vi "optical_grab2.vi"() -> ()   [LabVIEW 2025]
uses:
  <vilib>/vision/driver/NI_Vision_Acquisition_Software.lvlib
  <resource>/objmgr/imaqdx.rc
panel:
  in  "Stop 2":bool
  out "Time bw Frames":u32
  out "max value":u16
  out "Image Pixels (U16)":u16[][](array[numeric])
  out "Image Preview":T1(plugin-control)
  out "error out":errorcluster
  out "FPS":u32
  in  "Output Folder":path=path "../data/raw/test_6"
  in  "Stop":bool
  in  "Camera Name":refnum<k21> caption="IMAQdx Session"
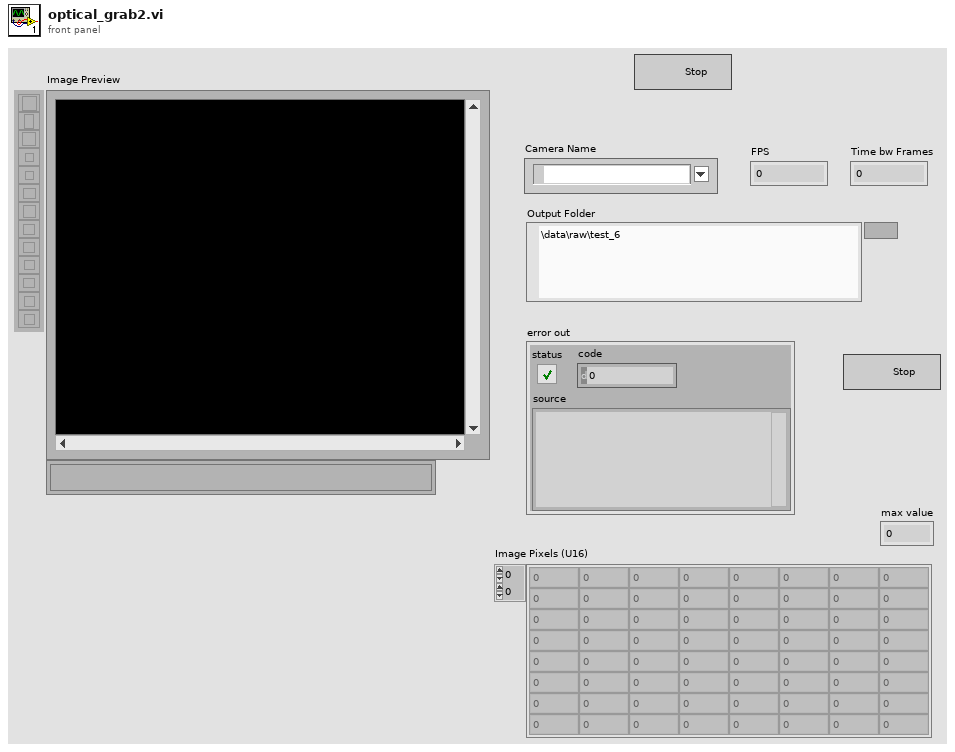
[diagram p1: front panel]
types:
  T1 = typedef "IMAQ Image.ctl" = refnum<image>
  T2 = typedef "Image Type" = u32
  T3 = typedef "IMAQdx.ctl" = refnum<k21>
  T4 = enum16{"big-endian, network order", "native, host order", "little-endian"}
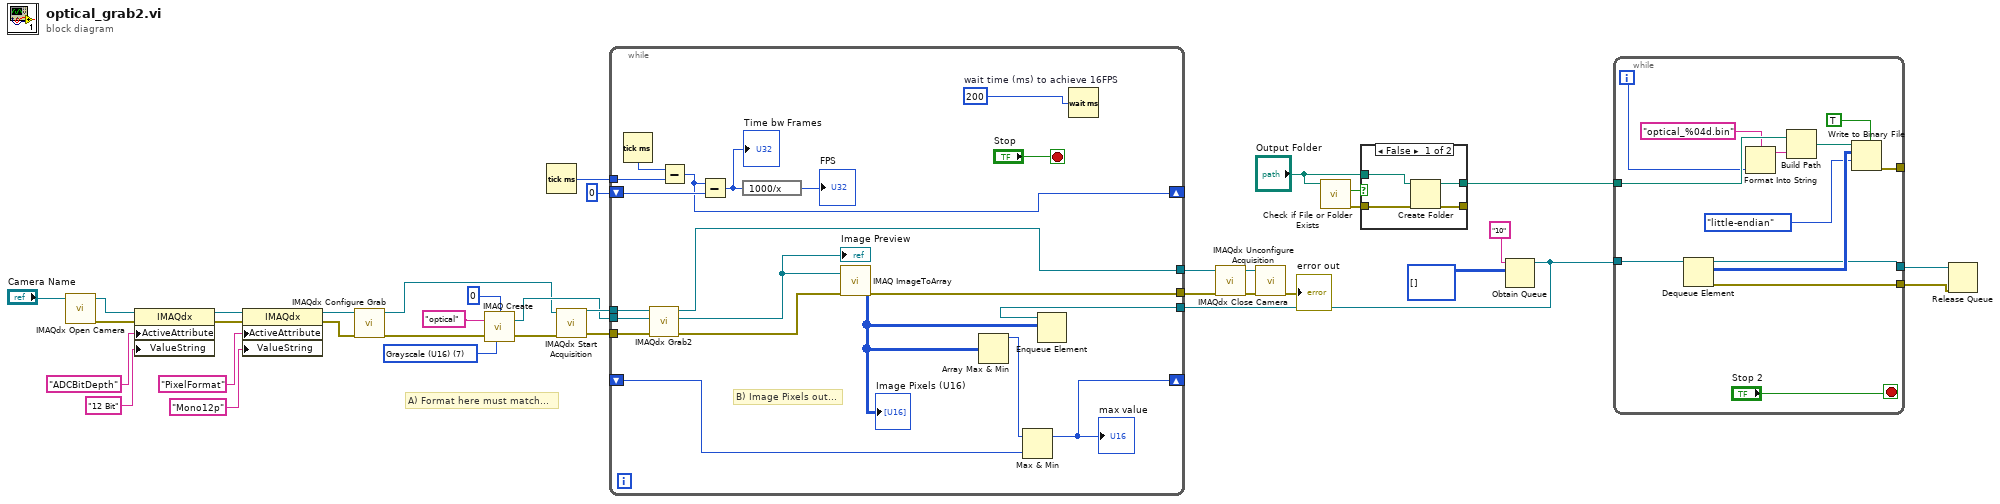
[diagram p0: block diagram]
diagram:
  w29 = T2 7 items=["Grayscale (U8)", "Grayscale (I16)", "Grayscale (SGL)", "Complex (CSG)", "RGB (U32)", "HSL (U32)", "RGB (U64)", "Grayscale (U16)"] ("Image Type")
  # "A) Format here must match..."
  n1 = call <vilib>:"IMAQdx Open Camera.vi"("Session In"="Camera Name") -> ("error out"=w25:errorcluster, "Session Out"=w26:T3)  [unwired: 9 in]
  n2 = property class="IMAQdx"(reference=w26, error in=w25, "ActiveAttribute"="ADCBitDepth", "ValueString"="12 Bit") -> (reference out=w16:T3, error out=w14:errorcluster)
  n3 = property class="IMAQdx"(reference=w16, error in=w14, "ActiveAttribute"="PixelFormat", "ValueString"="Mono12p" ("ActiveAttribute")) -> (reference out=w15:T3, error out=w13:errorcluster)
  n4 = call <vilib>:"IMAQdx Configure Grab.vi"("error in"=w13, "Session In"=w15) -> ("error out"=w20:errorcluster, "Session Out"=w19:T3)  [unwired: 8 in]
  n5 = call "IMAQ Create"("Border Size"=0, "Image Name"="optical", "Image Type"=w29, "error in (no error)"=w20) -> ("New Image"=w23:T1, "error out"=w22:errorcluster)  [unwired: 1 in]
  n6 = Tick Count (ms)() -> (millisecond timer value=w33:u32)
  n7 = call <vilib>:"IMAQdx Start Acquisition.vi"("error in"=w22, "Session In"=w19) -> ("error out"=w21:errorcluster, "Session Out"=w27:T3)  [unwired: 8 in]
  n8 = call <vilib>:"Check if File or Folder Exists.vi"("path"="Output Folder") -> ("error out"=w34:errorcluster, "file or folder exists?"=w36:bool)  [unwired: 8 in, 1 out]
  n9 = case shown="False" w36 {
    tunnel: "Output Folder" -> [w40 w42]
    tunnel: [w39 w42] -> w9
    tunnel: w34 -> [w38 w41]
    tunnel: [w37 w41] -> _
    frame False {
      n10 = Create Folder(path (use dialog)=w40, error in=w38) -> (created path=w39:path, error out=w37:errorcluster)  [unwired: 1 in, 1 out]
    }
    frame True {
    }
  }
  n11 = Obtain Queue(name (unnamed)="10", element data type=u16[][] [] ("Image Pixels (U16)")) -> (queue out=w4:refnum<queue>)  [unwired: 3 in, 2 out]
  n12 = while {
    tunnel: w33 -> [w61]
    shift-right: [w43] -> _
    shift-left: u32 0 -> [w60]
    tunnel: w27 -> [w58]
    tunnel: w23 -> [w57]
    tunnel: w21 -> [w56]
    shift-right: [w50] -> _
    shift-left: _ -> [w51]
    tunnel: [w47] -> w5
    tunnel: [w46] -> w8
    tunnel: w4 -> [w44]
    stop <- "Stop" stop-if-true
    w49 = u32 200  # wait time (ms) to achieve 16FPS
    # "B) Image Pixels out..."
    n13 = Tick Count (ms)() -> (millisecond timer value=w62:u32)
    n14 = call <vilib>:"IMAQdx Grab2.vi"("error in"=w56, "Image In"=w57, "Session In"=w58) -> ("error out"=w53:errorcluster, "Image Out"=w54:T1, "Session Out"=w46:T3)  [unwired: 5 in, 1 out]
    "Image Preview" <- w54
    n15 = Subtract(x=w62, y=w61) -> (x-y=w43:u32)
    n16 = Subtract(x=w43, y=w60) -> (x-y=w48:u32)
    "Time bw Frames" <- w48
    n17 = expression code="1000/x"(w48) -> (→"FPS":u32)
    n18 = call "IMAQ ImageToArray"("error in (no error)"=w53, "Image"=w54) -> ("Image Pixels (U16)"=w45:u16[][], "error out"=w47:errorcluster)  [unwired: 2 in, 3 out]
    "Image Pixels (U16)" <- w45
    n19 = Array Max & Min(array=w45) -> (max value=w52:u16)  [unwired: 3 out]
    n20 = Max & Min(x=w52, y=w51) -> (max(x,y)=w50:u16)  [unwired: 1 out]
    "max value" <- w50
    n21 = Enqueue Element(queue=w44, element=w45) -> ()  [unwired: 2 in, 3 out]
    n22 = Wait (ms)(milliseconds to wait=w49) -> ()  [unwired: 1 out]
  }
  n23 = call <vilib>:"IMAQdx Unconfigure Acquisition.vi"("error in"=w5, "Session In"=w8) -> ("error out"=w7:errorcluster, "Session Out"=w6:T3)  [unwired: 8 in]
  n24 = call <vilib>:"IMAQdx Close Camera.vi"("error in"=w7, "Session In"=w6) -> ("error out"=→"error out":errorcluster)  [unwired: 9 in]
  n25 = while {
    tunnel: [w75] -> _
    tunnel: w4 -> [w74]
    tunnel: w9 -> [w71]
    tunnel: [w64] -> w3
    tunnel: [w63] -> w1
    i -> [w66]
    stop <- "Stop 2" stop-if-true
    n26 = Dequeue Element(queue=w74) -> (queue out=w64:refnum<queue>, element=w72:u16[][], error out=w63:errorcluster)  [unwired: 2 in, 1 out]
    n27 = Format Into String(format string="optical_%04d.bin", w66) -> (resulting string=w69:string)  [unwired: 2 in, 1 out]
    n28 = Build Path(base path=w71, name or relative path=w69) -> (appended path=w70:path)
    n29 = Write to Binary File(file (use dialog)=w70, data=w72, 5:TRUE, 9:T4."little-endian" ("byte order (0:big-endian, network order)")) -> (error out=w75:errorcluster)  [unwired: 2 in, 2 out]
  }
  n30 = Release Queue(queue=w3, error in (no error)=w1) -> ()  [unwired: 1 in, 3 out]
